vi "Main.vi"() -> ()   [LabVIEW 2016, in "13.03 Robot.lvrbt"]
uses:
  13.03 Robot.lvrbt
  <vilib>/NXT/Block Support/NXT_InputPort.ctl
  <vilib>/NXT/Subs/ColorSensorColors.ctl
  <vilib>/NXT/Block Support/NXT_OutputPort.ctl
  <vilib>/NXT/Dual Mode Library/Sensors/EV3_Color_Color.vi
  <vilib>/NXT/Dual Mode Library/Display/drawText.vi
  <vilib>/NXT/NXTIO Xnodes/NXTIONodeSubVIs/NXTStopMotors.vi
  <vilib>/NXT/NXTIO Xnodes/NXTIONodeSubVIs/NXTMoveMotors.vi
  <vilib>/NXT/NXTIO Xnodes/AddressXNode/NXTIOAddress.xnode
  <vilib>/NXT/Subs/LVHSConnector.ctl
  <vilib>/NXT/NXTIO Xnodes/NXTIOXNode/NXTIO.xnode
  <vilib>/NXT/LegoClasses/BrickReference/BrickReference.lvclass
panel:
  in  "Speed":dbl
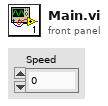
[diagram p1: front panel]
types:
  T1 = typedef "NXT_OutputPort.ctl" = u8
  T2 = typedef "ColorSensorColors.ctl" = enum16{"No Color", "Black", "Blue", "Green", "Yellow", "Red", "White", "Brown"}
  T3 = typedef "NXT_InputPort.ctl" = u32
  T4 = typedef "LVHSConnector.ctl" = refnum<class "BrickReference.lvclass">
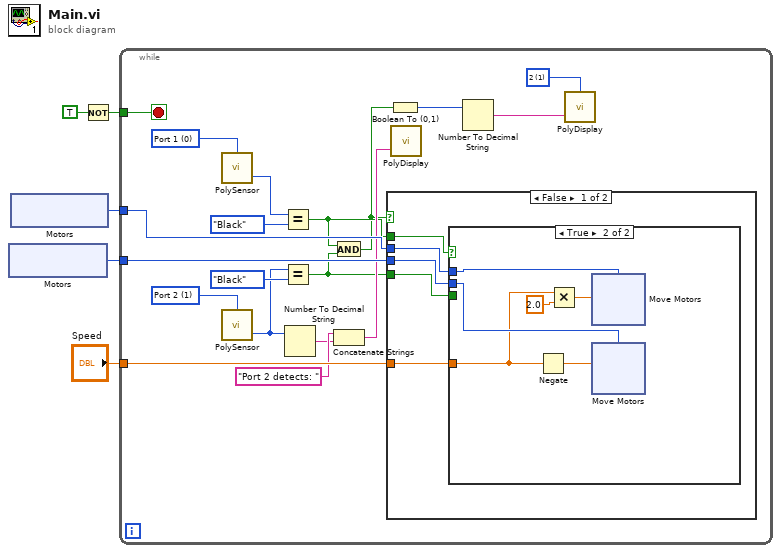
[diagram p0: block diagram]
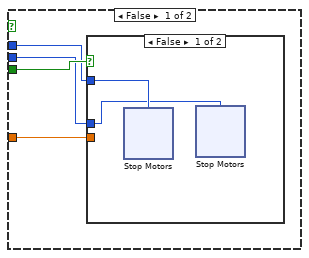
[diagram p2: hidden frame]
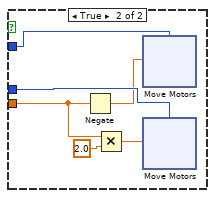
[diagram p3: hidden frame]
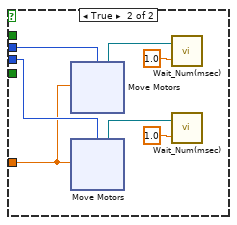
[diagram p4: hidden frame]
diagram:
  n1 = xnode "Motors"() -> ("Motor"=w5:T1)
  n2 = xnode "Motors"() -> ("Motor"=w4:T1)
  n3 = Not(x=TRUE) -> (.not. x?=w1:bool)
  n4 = while {
    tunnel: w5 -> [w20]
    tunnel: w4 -> [w19]
    tunnel: "Speed" -> [w18]
    tunnel: w1 -> [w17]
    stop <- w17 stop-if-true
    w9 = i16 1 items=["1", "2", "3", "4", "5", "6", "7", "8", "9", "10", "11", "12"] ("Line")
    w22 = T3 1 items=["Port 1", "Port 2", "Port 3", "Port 4"] ("Port (Port 1)")
    w24 = T3 0 items=["Port 1", "Port 2", "Port 3", "Port 4"] ("Port (Port 1)")
    n5 = call-poly <vilib>:"PolySensor.vi"("Port (Port 1)"=w24) -> ("Detected Color"=w23:T2)  [unwired: 2 in, 1 out]
    n6 = call-poly <vilib>:"PolySensor.vi"("Port (Port 1)"=w22) -> ("Detected Color"=w14:T2)  [unwired: 2 in, 1 out]
    n7 = Equal?(x=w23, y=ColorSensorColors."Black" ("Detected Color")) -> (x = y?=w8:bool)
    n8 = Equal?(x=w14, y=ColorSensorColors."Black" ("Detected Color")) -> (x = y?=w6:bool)
    n9 = Number To Decimal String(number=w14) -> (decimal integer string=w13:string)  [unwired: 1 in]
    n10 = And(x=w8, y=w6) -> (x .and. y?=w7:bool)
    n11 = Concatenate Strings("Port 2 detects: " ("string"), w13) -> (w12:string)
    n12 = case shown="False" w7 {
      tunnel: w20 -> [w26 w92]
      tunnel: w19 -> [w28 w91]
      tunnel: w18 -> [w27 w90]
      tunnel: w8 -> [w29 _]
      tunnel: w6 -> [w25 _]
      frame False {
        n13 = case shown="True" w29 {
          tunnel: w28 -> [w30 w71]
          tunnel: w27 -> [w31 w67]
          tunnel: w26 -> [w32 w69]
          tunnel: w25 -> [w33 _]
          frame False {
            n14 = case shown="False" w33 {
              tunnel: w32 -> [w34 w51]
              tunnel: w31 -> [_ w47]
              tunnel: w30 -> [w35 w50]
              frame False {
                n15 = xnode "Stop Motors"("Motors"=w35) -> ()  [unwired: 1 in, 1 out]
                n16 = xnode "Stop Motors"("Motors"=w34) -> ()  [unwired: 1 in, 1 out]
              }
              frame True {
                n17 = Negate(x=w47) -> (-x=w49:dbl)
                n18 = Multiply(x=w47, y=2.0) -> (x*y=w46:dbl)
                n19 = xnode "Move Motors"("Power/Speed 1"=w49, "Motors"=w50) -> ()  [unwired: 1 in, 1 out]
                n20 = xnode "Move Motors"("Power/Speed 1"=w46, "Motors"=w51) -> ()  [unwired: 1 in, 1 out]
              }
            }
          }
          frame True {
            n21 = Negate(x=w67) -> (-x=w70:dbl)
            n22 = Multiply(x=w67, y=2.0) -> (x*y=w66:dbl)
            n23 = xnode "Move Motors"("Power/Speed 1"=w66, "Motors"=w71) -> ()  [unwired: 1 in, 1 out]
            n24 = xnode "Move Motors"("Power/Speed 1"=w70, "Motors"=w69) -> ()  [unwired: 1 in, 1 out]
          }
        }
      }
      frame True {
        n25 = xnode "Move Motors"("Power/Speed 1"=w90, "Motors"=w91) -> ("NXT/EV3"=w86:T4)  [unwired: 1 in]
        n26 = xnode "Move Motors"("Power/Speed 1"=w90, "Motors"=w92) -> ("NXT/EV3"=w87:T4)  [unwired: 1 in]
        n27 = call <vilib>:"Wait_Num(msec).vi"("Time (100 msec)"=sgl 1.0 ("Time (1 sec)"), "NXT/EV3"=w86) -> ()  [unwired: 2 in, 1 out]
        n28 = call <vilib>:"Wait_Num(msec).vi"("Time (100 msec)"=sgl 1.0 ("Time (1 sec)"), "NXT/EV3"=w87) -> ()  [unwired: 2 in, 1 out]
      }
    }
    n29 = Boolean To (0,1)(Boolean=w7) -> (0, 1=w11:i16)
    n30 = call-poly <vilib>:"PolyDisplay.vi"("Text"=w12) -> ()  [unwired: 3 in, 1 out]
    n31 = Number To Decimal String(number=w11) -> (decimal integer string=w10:string)  [unwired: 1 in]
    n32 = call-poly <vilib>:"PolyDisplay.vi"("Text"=w10, "Line"=w9) -> ()  [unwired: 2 in, 1 out]
  }
